vi "3D get Target Position.vi"(8 "error in (no error)":errorcluster caption="에러 입력(에러 없음)", 10 "Antenna Pol":enum16{"H", "V"}(ring), 11 "Instrument Manager 입력":refnum<class "Instrument Manager.lvclass">) -> (0 "error out":errorcluster caption="에러 출력", 2 "Target Position (deg)":dbl format="%#_13g", 3 "Instrument Manager 출력":refnum<class "Instrument Manager.lvclass">)   [LabVIEW 2023, in "Instrument Manager.lvclass"]
uses:
  Instrument Manager.lvclass
  Instrument Manager.lvclass/Instrument Manager.ctl
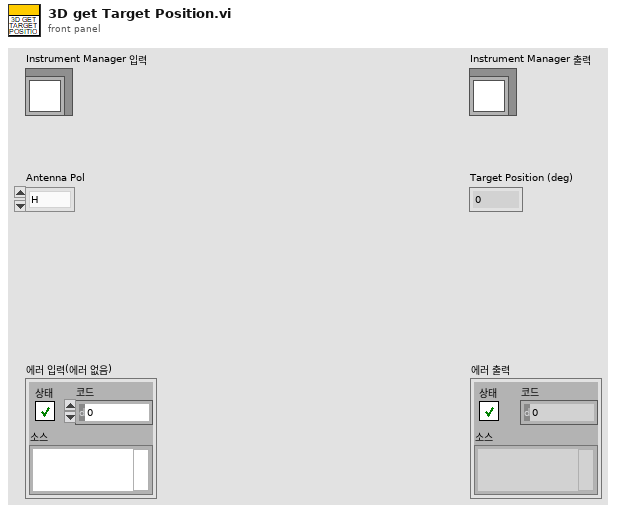
[diagram p1: front panel]
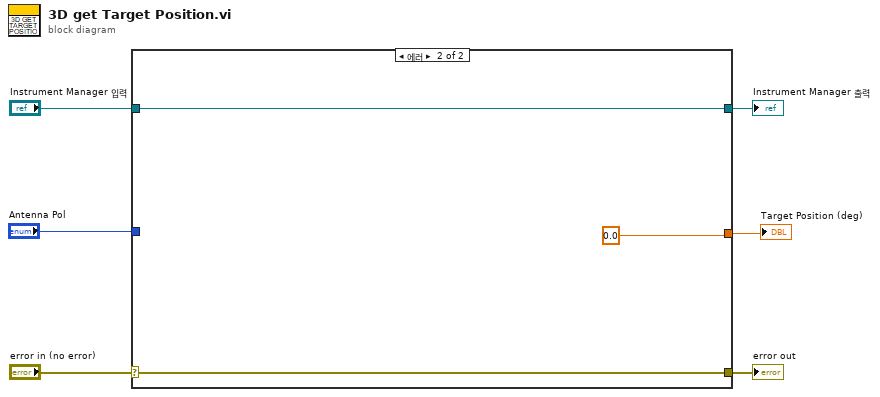
[diagram p0: block diagram]
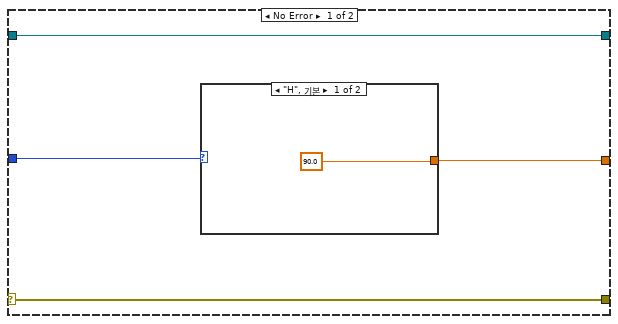
[diagram p2: hidden frame]
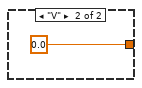
[diagram p3: hidden frame]
diagram:
  n1 = case shown="에러" "error in (no error)" {
    selector: "error in (no error)" -> [w9 w15]
    tunnel: [w9 w15] -> w5
    tunnel: [w10 w14] -> w3
    tunnel: "Instrument Manager 입력" -> [w10 w14]
    tunnel: "Antenna Pol" -> [w8 _]
    tunnel: [w7 0.0 ("Target Position (deg)")] -> w1
    frame No Error {
      n2 = case shown="\"H\", 기본" w8 {
        tunnel: [90.0 ("Target Position (deg)") 0.0 ("Target Position (deg)")] -> w7
        frame "H", Default {
        }
        frame "V" {
        }
      }
    }
    frame Error {
    }
  }
  "error out" <- w5
  "Instrument Manager 출력" <- w3
  "Target Position (deg)" <- w1
